vi "editDialog.vi"(0 "reference":refnum<class "InterfaceNode.lvclass">, 1 "insidePackageNode":bool, 5 "error in (no error)":errorcluster) -> (14 "reference out":refnum<class "InterfaceNode.lvclass">, 15 "changeConnection":T1, 16 "cancel":bool, 19 "error out":errorcluster)   [LabVIEW 2020, in "InterfaceNode.lvclass"]
doc: "Edit Dialog"
uses:
  <resource>/Framework/Providers/Open_GDS/UML/InterfaceNode_class/InterfaceNode.lvclass
  C:/Program Files (x86)/National Instruments/LabVIEW 2020/resource/Framework/Providers/Open_GDS/UML/ClassNode_class/ClassNode.lvclass
  C:/Program Files (x86)/National Instruments/LabVIEW 2020/resource/Framework/Providers/Open_GDS/UML/AbstractNode_class/AbstractNode.lvclass
  <resource>/Framework/Providers/Open_GDS/UML/AbstractNode_class/private/NodeConnectionStatsType.ctl
  <resource>/Framework/Providers/Open_GDS/UML/ContextHelp/ContextHelp_HelpTexts.ctl
  <resource>/Framework/Providers/Open_GDS/UML/MultiLineString_class/MultiLineString.lvclass
  <resource>/Framework/Providers/Open_GDS/UML/AbstractNode_class/AbstractNode.lvclass
  <resource>/Framework/Providers/Open_GDS/UML/ClassNode_class/ClassNode.lvclass
panel:
  in  "ShowMethods":bool caption="Show Methods"
  out "RelText":string="Relative path used"
  in  "ClassPath":path caption="LvClassPath(Optional)"
  in  "Help":bool
  in  "AddMethod":bool
  in  "connection":bool caption="Connect to Package"
  in  "Interface Name":string
  in  "Cancel Button":bool
  in  "OK Button":bool
  in  "Methods":string
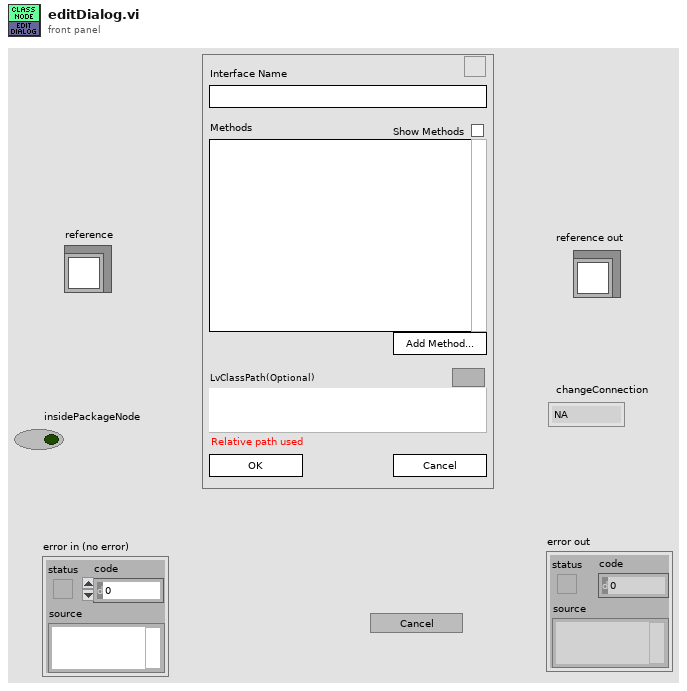
[diagram p1: front panel]
types:
  T1 = typedef "AbstractNode.lvclass/NodeConnectionStatsType.ctl" = enum16{"NA", "Connect", "DisConnect"}
  T2 = typedef "ContextHelp_HelpTexts.ctl" = enum16{"None(Hide)", "Default", "Help", "Welcome", "GettingStarted", "ClassDiagram_Help", "SequenceDiagram_Help", "UseCaseDiagram_Help", "BSelect", "BClass", "BInterface", "BPackage", "BNote", "BDependency", "BInheritance", "BInterfaceImplementation", "BAssociation", "BAggregation", "BCompAggregation", "BNoteConnector", "BObject", "BActionBar", "BCall", "BSystem", "BActor", "BUseCase", "BGeneralization", "BIncludes", "BExtends", "BUseCaseDiagramAssociation", "ClassRelationshipEdge editDialog_Bent Style", "ClassRelationshipEdge editDialog_RelationType", "ClassRelationshipEdge editDialog_Reverse association", "ClassRelationshipEdge editDialog_Start label", "ClassRelationshipEdge editDialog_Middle label", "ClassRelationshipEdge editDialog_End label", "UMLEditor reversedEngineering_Pathes", "ReversedEngineering StateReverseDialog_Help", "ReversedEngineering StateQueuedSettings_Help", "UMLEditor reversedEngineering_AddTopVIs", "UMLEditor reversedEngineering_AddClasses", "UMLEditor reversedEngineering_AddDirs", "UMLEditor reversedEngineering_Recursively", "UMLEditor reversedEngineering_Remove", "UMLEditor reversedEngineering_ClearList", "UMLEditor reversedEngineering_HideSubAss", "UMLEditor reversedEngineering_CreateTypes", "UMLEditor reversedEngineering_OnlyInheritance", "UMLEditor reversedEngineering_CreateApplication", "UMLEditor reversedEngineering_OK", "UMLEditor reversedEngineering_Cancel", "UMLEditor reversedEngineering_Help", "UMLEditor createWizardScriptFile_ScriptfilePath", "UMLEditor createWizardScriptFile_ClassPath", "UMLEditor createWizardScriptFile_Use", "UMLEditor createWizardScriptFile_PrivateDirName", "UMLEditor createWizardScriptFile_DirAppend", "UMLEditor createWizardScriptFile_Separator Character", "UMLEditor createWizardScriptFile_OK", "UMLEditor createWizardScriptFile_Cancel", "UMLEditor createWizardScriptFile_Help", "ClassNode editDialog_Class Name", "InterfaceNode editDialog_Class Name", "ClassNode editDialog_Attribute", "ClassNode editDialog_Methods", "InterfaceNode editDialog_Methods", "ClassNode editDialog_connection", "InterfaceNode editDialog_connection", "ClassNode editDialog_StereoType", "ClassNode editDialog_ShowAttrib", "ClassNode editDialog_ShowMethods", "ClassNode editDialog_ClassPath", "ClassNode editDialog_AddAttribute", "ClassNode editDialog_AddMethod", "InterfaceNode editDialog_AddMethod", "ClassNode AttributeGuide_AttributeName", "ClassNode AttributeGuide_Array?", "ClassNode AttributeGuide_Data Type", "ClassNode AttributeGuide_RefName", "ClassNode AttributeGuide_Preview", "ClassNode AttributeGuide_OK", "ClassNode AttributeGuide_Cancel", "ClassNode MethodGuide_Visibility", "ClassNode MethodGuide_Method Name", "ClassNode MethodGuide_Preview", "ClassNode MethodGuide_OK", "ClassNode MethodGuide_Cancel", "CallNode EditCallProperties_AllButtons", "ObjectNode EditObjectlProperties_AllButtons", "ActorNode EditActorProperties_AllButtons", "UseCaseRelationshipNode EditUseCaselProperties_AllButtons", "UseCaseNode EditUseCaselProperties_AllButtons", "SystemNode EditSystemProperties_AllButtons", "ReversedEngineering UpdateAttributes_AllButtons", "StateNode editDialog_AllButtons", "StateTransition editDialog_AllButtons", "ArrangeNodes Main_Picture", "ArrangeNodes Main_Zoom", "ArrangeNodes Main_Auto Zoom", "ArrangeNodes Main_shorten", "ArrangeNodes Main_Min Length", "ArrangeNodes Main_Max Length", "ArrangeNodes Main_increase", "ArrangeNodes Main_decrease", "ArrangeNodes Main_Shake", "ArrangeNodes Main", "BState", "BInitialState", "BFinalState", "BStateTransition", "StateDiagram_Help", "StateDiagram_PropertiesAllButtons", "ReversedEngineering StateReverseDialog_ClearStates", "ReversedEngineering StateReverseDialog_UseQueuedStateMachines", "ReversedEngineering StateReverseDialog_QueuedSettings", "ReversedEngineering StateReverseDialog_SearchForVIs", "ReversedEngineering StateReverseDialog_SearchCriteria", "OptionsDialog_ClassBasePath", "OptionsDialog_VIPath", "OptionsDialog_ApplicationPath", "OptionsDialog_WizDir", "OptionsDialog_IniFilePath", "OptionsDialog_DefineColors", "OptionsDialog_Help", "OptionsDialog_CreateTypes", "ClassRelationshipEdge editDialog_SplitWire"}
  T3 = enum16{"None", "TYPE", "ENUM", "ABSTRACT", "ACTOR", "GUI", "SINGLETON", "SIGNAL", "BOUNDARY", "ENTITY", "CONTROL", "LEGACY", "APPLICATION", "VI", "LVLIB"}
  T4 = typedef "ClassNode.lvclass/ObjectAttributes.ctl" = cluster{"midHeight":dbl, "botHeight":dbl, "name":refnum<class "MultiLineString.lvclass">, "attributes":refnum<class "MultiLineString.lvclass">, "methods":refnum<class "MultiLineString.lvclass">, "DEFAULT_COMPARTMENT_HEIGHT":i32, "DEFAULT_WIDTH":i32, "DEFAULT_HEIGHT":i32, "showMethods":bool, "showAttributes":bool, "ClassPath":path}
  T5 = typedef "AbstractNode.lvclass/ObjectAttributes.ctl" = cluster{"parent":refnum<class "AbstractNode.lvclass">, "children":refnum<class "AbstractNode.lvclass">[], "Hidden":bool}
  T6 = typedef "ContextHelp_ShowType.ctl" = cluster{"Header":string, "Picture":picture, "Text":string}
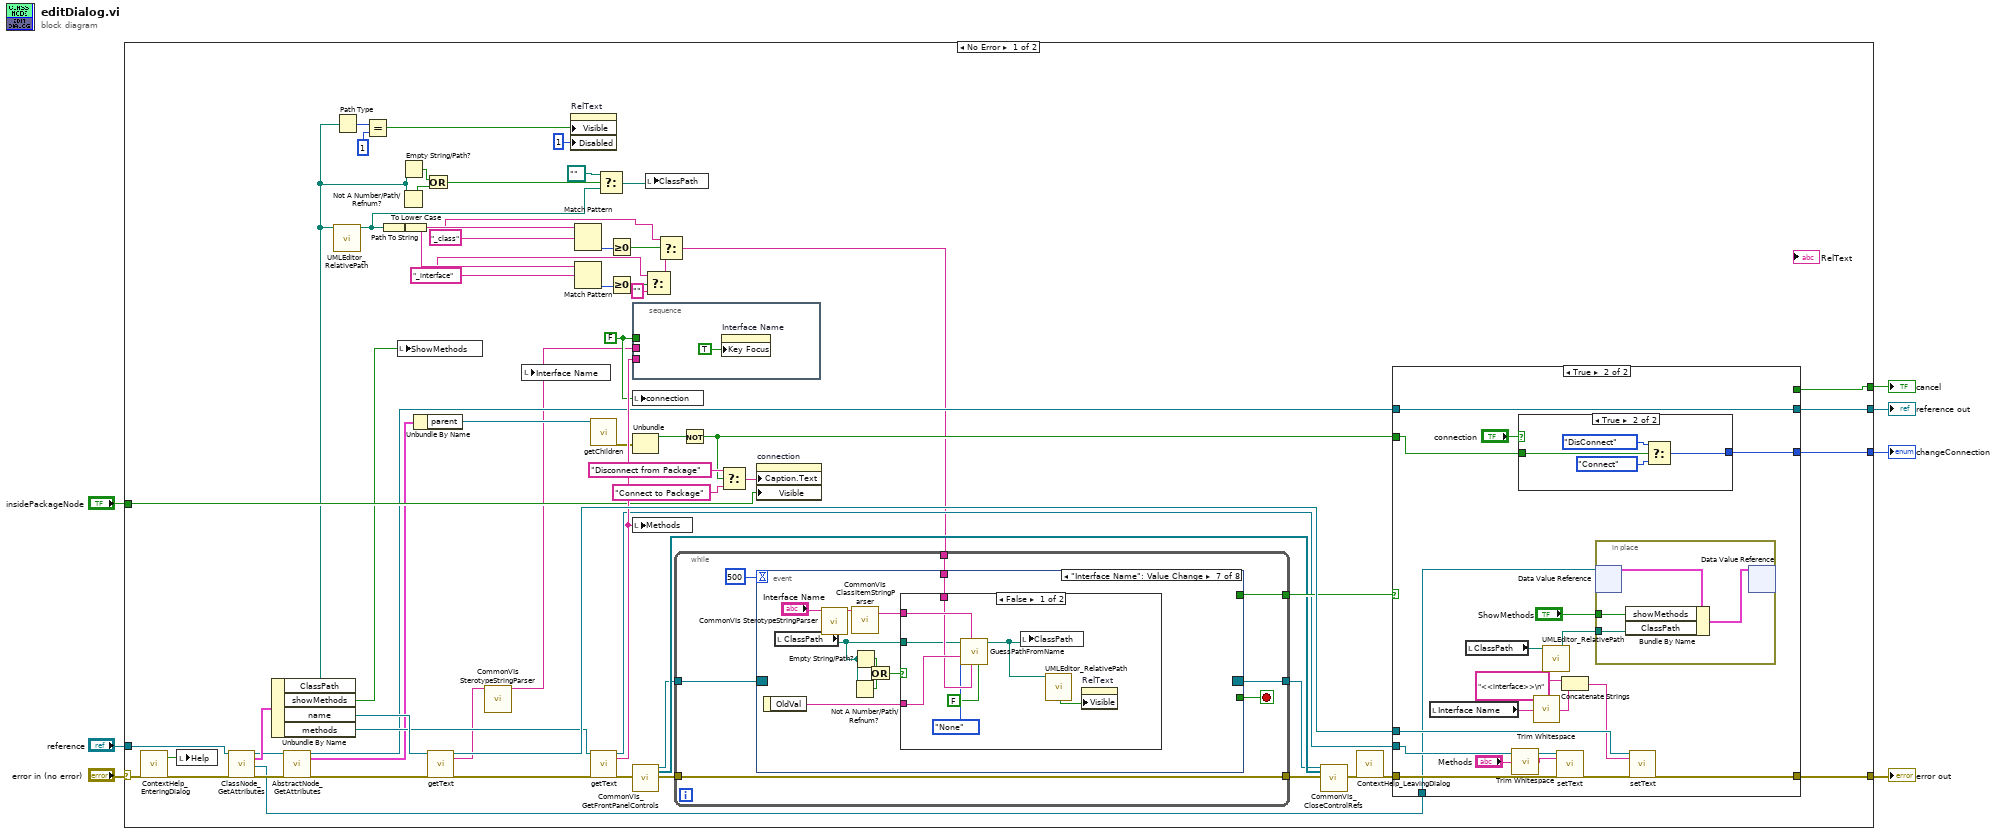
[diagram p0: block diagram]
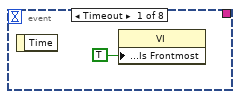
[diagram p2: hidden frame]
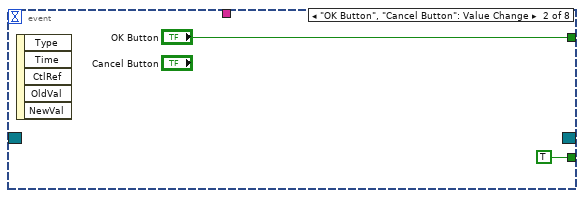
[diagram p3: hidden frame]
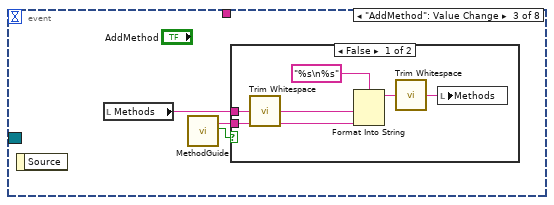
[diagram p4: hidden frame]
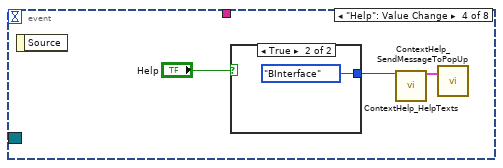
[diagram p6: hidden frame]
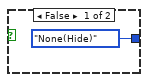
[diagram p7: hidden frame]
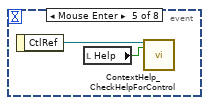
[diagram p8: hidden frame]
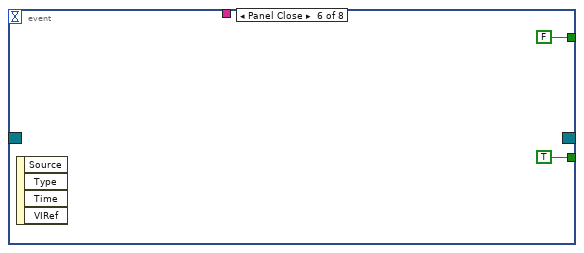
[diagram p9: hidden frame]
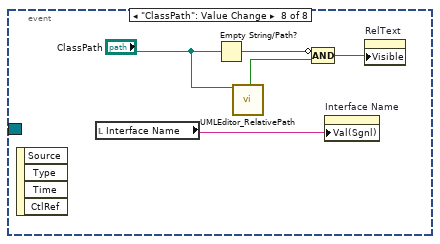
[diagram p11: hidden frame]
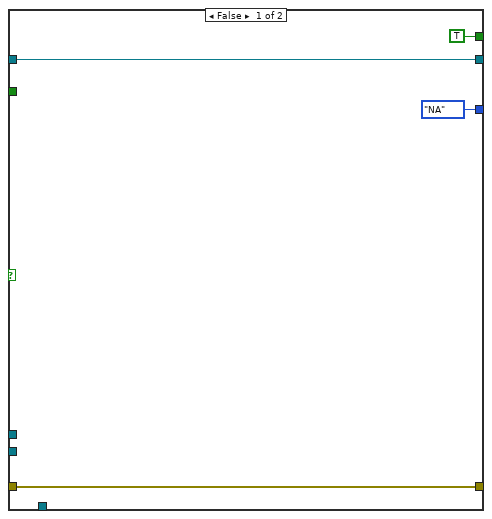
[diagram p12: hidden frame]
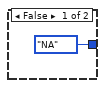
[diagram p13: hidden frame]
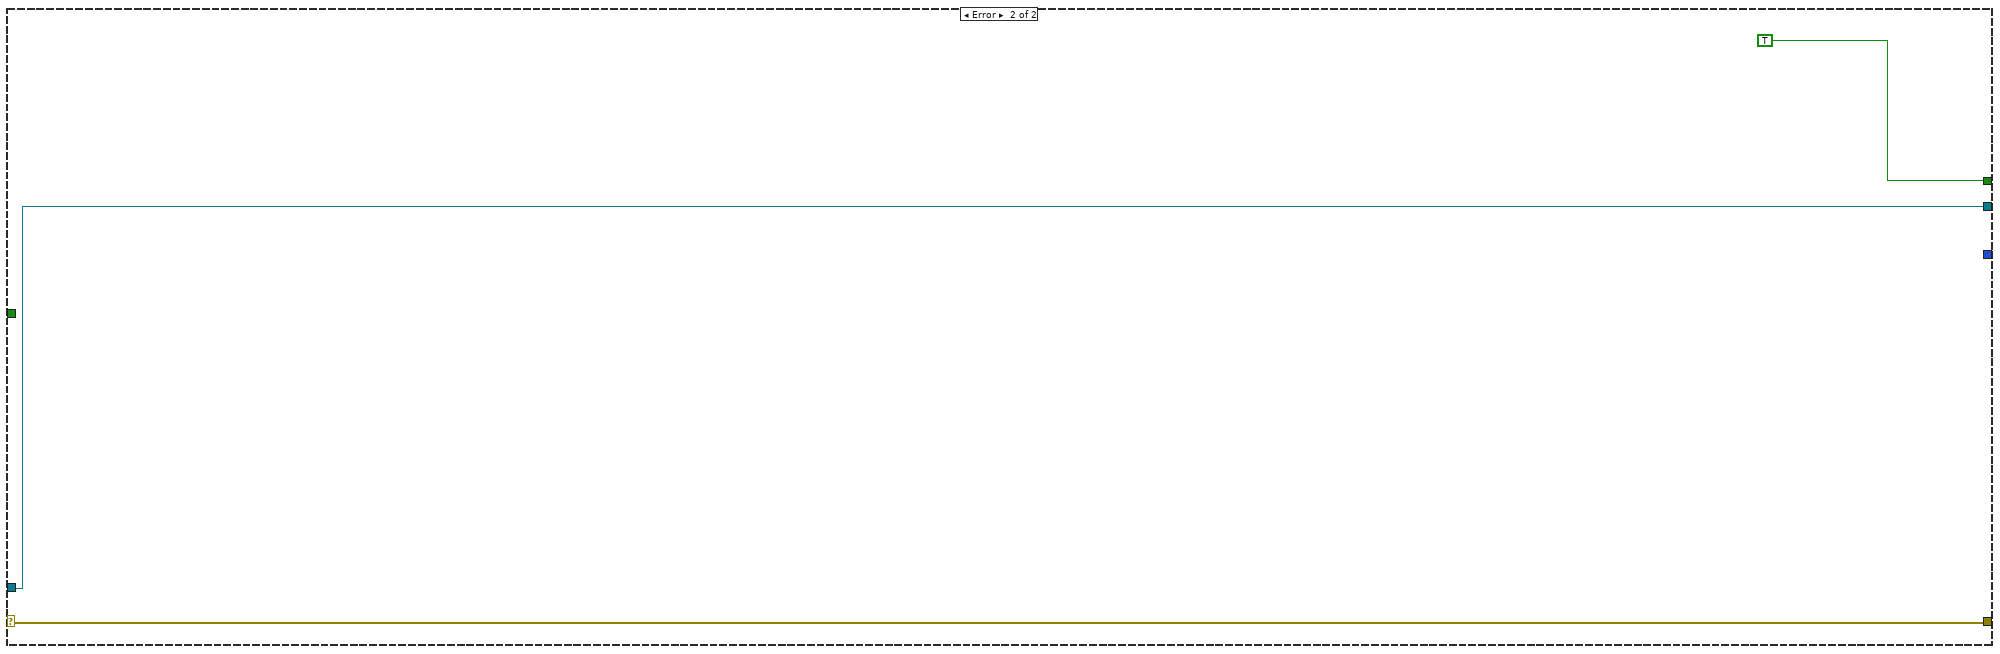
[diagram p14: hidden frame]
diagram:
  n1 = case shown="No Error" "error in (no error)" {
    selector: "error in (no error)" -> [w36 w156]
    tunnel: "reference" -> [w69 w157]
    tunnel: [w71 w156] -> w5
    tunnel: [w70 w157] -> w4
    tunnel: [w61 _] -> w3
    tunnel: "insidePackageNode" -> [w57 _]
    tunnel: [w55 TRUE ("Key Focus")] -> w1
    frame No Error {
      w14 = "_interface" ("regular expression")
      w15 = "_class" ("regular expression")
      w56 = FALSE ("connection")
      n2 = call <resource>:"ContextHelp_EnteringDialog.vi"("error in (no error)"=w36) -> ("HelpStatus"=w53:bool, "error out"=w35:errorcluster)  [unwired: 2 in, 15 out]
      n3 = local write "Help"(w53) -> ()
      n4 = call <resource>:"ClassNode_GetAttributes.vi"("reference in"=w69, "error in (no error)"=w35) -> ("reference out"=w42:refnum<class "InterfaceNode.lvclass">, "Data"=w43:T4, "DataRef"=w11:refnum<data-value>, "error out"=w41:errorcluster)  [unwired: 14 in]
      n5 = Unbundle By Name(w43) -> ("ClassPath"=w22:path, "showMethods"=w8:bool, "name"=w66:refnum<class "MultiLineString.lvclass">, "methods"=w64:refnum<class "MultiLineString.lvclass">)
      n6 = call <resource>:"AbstractNode_GetAttributes.vi"("reference in"=w42, "error in (no error)"=w41) -> ("reference out"=w39:refnum<class "InterfaceNode.lvclass">, "Data"=w38:T5, "error out"=w40:errorcluster)  [unwired: 14 in, 1 out]
      n7 = call <resource>:"UMLEditor_RelativePath.vi"("Path In"=w22) -> ("ConvertToAbsolutePath(If possible)"=w19:path)  [unwired: 1 in, 17 out]
      n8 = Path Type(1:w22) -> (0:w32:i16)
      n9 = Equal?(x=w32, y=i16 1) -> (x = y?=w30:bool)
      n10 = Path To String(path=w19) -> (string=w23:string)
      n11 = local write "ShowMethods"(w8) -> ()
      n12 = Not A Number/Path/Refnum?(number/path/refnum=w22) -> (NaN/Path/Refnum?=w28:bool)
      n13 = Empty String/Path?(string/path=w22) -> (empty?=w29:bool)
      n14 = To Lower Case(string=w23) -> (all lower case string=w20:string)
      n15 = Unbundle By Name(w38) -> ("parent"=w45:refnum<class "AbstractNode.lvclass">)
      n16 = Or(x=w29, y=w28) -> (x .or. y?=w26:bool)
      n17 = call-dynamic "getText.vi"("reference"=w66, "error in (no error)"=w40) -> ("reference out"=w68:refnum<class "MultiLineString.lvclass">, "text"=w10:string, "error out"=w62:errorcluster)  [unwired: 15 in]
      n18 = call <resource>:"CommonVIs SterotypeStringParser.vi"("SterotypeStringIn"=w10) -> ("Name"=w9:string)  [unwired: 18 out]
      n19 = local write "Interface Name"(w9) -> ()
      n20 = property on="RelText" class="Str"("Visible"=w30, "Disabled"=u8 1) -> ()  [unwired: 2 in, 2 out]
      n21 = Match Pattern(string=w20, regular expression=w15) -> (offset past match=w24:i32)  [unwired: 1 in, 3 out]
      n22 = Match Pattern(string=w20, regular expression=w14) -> (offset past match=w21:i32)  [unwired: 1 in, 3 out]
      n23 = call-dynamic "getChildren.vi"("reference"=w45) -> ("error out"=w47:errorcluster)  [unwired: 15 in, 3 out]
      n24 = call-dynamic "getText.vi"("reference"=w64, "error in (no error)"=w62) -> ("reference out"=w63:refnum<class "MultiLineString.lvclass">, "text"=w65:string, "error out"=w37:errorcluster)  [unwired: 15 in]
      n25 = Select(t=path "", s=w26, f=w19) -> (s? t:f=w25:path)
      n26 = Greater Or Equal To 0?(x=w24) -> (x >= 0?=w18:bool)
      n27 = Greater Or Equal To 0?(x=w21) -> (x >= 0?=w16:bool)
      n28 = stacked-sequence {
        tunnel: w9 -> [_]
        tunnel: w65 -> [_]
        tunnel: w56 -> [_]
        frame #0 {
          n29 = property on="Interface Name" class="Str"("Key Focus"=TRUE) -> ()  [unwired: 2 in, 2 out]
        }
      }
      n30 = local write "connection"(w56) -> ()
      n31 = Unbundle(w47) -> ("status"=w46:bool)  [unwired: 2 out]
      n32 = local write "Methods"(w65) -> ()
      n33 = call <resource>:"CommonVIs_GetFrontPanelControls.vi"("error in (no error)"=w37) -> ("Event Registration Refnum"=w49:refnum<event-registration>, "ControlRefs"=w50:refnum<vi>[], "error out"=w54:errorcluster)  [unwired: 1 in, 15 out]
      n34 = local write "ClassPath"(w25) -> ()
      n35 = Select(t=w14, s=w16, f="") -> (s? t:f=w17:string)
      n36 = Select(t=w15, s=w18, f=w17) -> (s? t:f=w12:string)
      n37 = while {
        tunnel: [w78] -> w67
        tunnel: [w75] -> w52
        tunnel: w54 -> [w75]
        tunnel: w49 -> [w74]
        tunnel: [w73] -> w48
        tunnel: w12 -> [w72]
        stop <- w76 stop-if-true
        n38 = event shown="[6] \"Interface Name\": Value Change" {
          selector: w74 -> [_ _ _ _ _ _ _ _]
          dyn-events: [_ _ _ _ _ _ _ _] -> w73
          timeout: 500 -> [_ _ _ _ _ _ _ _]
          tunnel: [_ "OK Button" _ _ _ FALSE ("OK Button") _ _] -> w78
          tunnel: [_ TRUE _ _ _ TRUE ("Front Panel Window:Is Frontmost") _ _] -> w76
          tunnel: w72 -> [_ _ _ _ _ _ w104 _]
          event Timeout {
            n39 = event-data() -> ()  [unwired: 2 out]
            n40 = property class="VI"("Front Panel Window:Is Frontmost"=TRUE) -> ()  [unwired: 2 in, 2 out]
          }
          event "OK Button", "Cancel Button": Value Change {
            n41 = event-data() -> ()  [unwired: 6 out]
          }
          event "AddMethod": Value Change {
            n42 = event-data() -> ()  [unwired: 2 out]
            n43 = local read "Methods"() -> (w84:string)
            n44 = call <resource>:"MethodGuide.vi"() -> ("Preview"=w83:string, "Canceled"=w82:bool)  [unwired: 1 in, 17 out]
            n45 = case shown="False" w82 {
              tunnel: w84 -> [w90 _]
              tunnel: w83 -> [w87 _]
              frame False {
                n46 = call <vilib>:"Trim Whitespace.vi"("string"=w90) -> ("trimmed string"=w88:string)  [unwired: 1 in]
                n47 = Format Into String(format string="%s\n%s", w88, w87) -> (resulting string=w86:string)  [unwired: 2 in, 1 out]
                n48 = call <vilib>:"Trim Whitespace.vi"("string"=w86) -> ("trimmed string"=w85:string)  [unwired: 1 in]
                n49 = local write "Methods"(w85) -> ()
              }
              frame True {
              }
            }
          }
          event "Help": Value Change {
            n50 = event-data() -> ()  [unwired: 2 out]
            n51 = case shown="True" "Help" {
              tunnel: [ContextHelp_HelpTexts."None(Hide)" ("HelpText") ContextHelp_HelpTexts."BInterface" ("HelpText")] -> w92
              frame False {
              }
              frame True {
              }
            }
            n52 = call <resource>:"ContextHelp_HelpTexts.vi"("HelpText (enum or string)"=w92) -> ("HelpOut"=w93:T6)  [unwired: 18 out]
            n53 = call <resource>:"ContextHelp_SendMessageToPopUp.vi"("PopUpMessage"=w93) -> ()  [unwired: 2 in, 17 out]
          }
          event Mouse Enter {
            n54 = event-data() -> ("CtlRef"=w97:refnum<vi>)  [unwired: 1 out]
            n55 = local read "Help"() -> (w96:bool)
            n56 = call <resource>:"ContextHelp_CheckHelpForControl.vi"("Ctl Refnum"=w97, "Help"=w96) -> ()  [unwired: 1 in, 17 out]
          }
          event Panel Close {
            n57 = event-data() -> ()  [unwired: 5 out]
          }
          event "Interface Name": Value Change {
            n58 = event-data() -> ("OldVal"=w105:string)  [unwired: 1 out]
            n59 = local read "ClassPath"() -> (w101:path)
            n60 = call <resource>:"CommonVIs SterotypeStringParser.vi"("SterotypeStringIn"="Interface Name") -> ("Name"=w108:string)  [unwired: 18 out]
            n61 = Not A Number/Path/Refnum?(number/path/refnum=w101) -> (NaN/Path/Refnum?=w103:bool)
            n62 = call <resource>:"CommonVIs ClassItemStringParser.vi"("ClassItemNameIn"=w108) -> ("Name"=w106:string)  [unwired: 18 out]
            n63 = Empty String/Path?(string/path=w101) -> (empty?=w102:bool)
            n64 = Or(x=w102, y=w103) -> (x .or. y?=w100:bool)
            n65 = case shown="False" w100 {
              tunnel: w106 -> [w116 _]
              tunnel: w105 -> [w115 _]
              tunnel: w104 -> [w114 _]
              tunnel: w101 -> [w109 _]
              frame False {
                n66 = call <resource>:"GuessPathFromName.vi"("Don'tAppendName"=FALSE, "FolderSuffix"=w114, "NewName"=w116, "OldName"=w115, "Stereo Type"=T3."None", "PathIn"=w109) -> ("File Path"=w112:path)  [unwired: 5 in]
                n67 = local write "ClassPath"(w112) -> ()
                n68 = call <resource>:"UMLEditor_RelativePath.vi"("Path In"=w112) -> ("ConvertedToARelativePath"=w111:bool)  [unwired: 1 in, 17 out]
                n69 = property on="RelText" class="Str"("Visible"=w111) -> ()  [unwired: 2 in, 2 out]
              }
              frame True {
              }
            }
          }
          event "ClassPath": Value Change {
            n70 = event-data() -> ()  [unwired: 5 out]
            n71 = local read "Interface Name"() -> (w117:string)
            n72 = Empty String/Path?(string/path="ClassPath") -> (empty?=w121:bool)
            n73 = call <resource>:"UMLEditor_RelativePath.vi"("Path In"="ClassPath") -> ("ConvertedToARelativePath"=w120:bool)  [unwired: 1 in, 17 out]
            n74 = Compound Arithmetic op=AND(invert w121, w120) -> (w118:bool)
            n75 = property on="Interface Name" class="Str"("Val(Sgnl)"=w117) -> ()  [unwired: 2 in, 2 out]
            n76 = property on="RelText" class="Str"("Visible"=w118) -> ()  [unwired: 2 in, 2 out]
          }
        }
      }
      n77 = Not(x=w46) -> (.not. x?=w44:bool)
      n78 = Select(t="Disconnect from Package", s=w44, f="Connect to Package") -> (s? t:f=w60:string)
      n79 = property on="connection" class="Bool (strict)"("Caption.Text"=w60, "Visible"=w57) -> ()  [unwired: 2 in, 2 out]
      n80 = call <resource>:"CommonVIs_CloseControlRefs.vi"("Event Registration Refnum"=w48, "ControlRefs"=w50, "error in (no error)"=w52) -> ("error out"=w51:errorcluster)  [unwired: 16 out]
      n81 = call <resource>:"ContextHelp_LeavingDialog.vi"("error in (no error)"=w51) -> ("error out"=w34:errorcluster)  [unwired: 2 in, 16 out]
      n82 = case shown="True" w67 {
        tunnel: [w124 w139] -> w71
        tunnel: [w125 w140] -> w70
        tunnel: w39 -> [w125 w140]
        tunnel: w68 -> [_ w144]
        tunnel: w63 -> [_ w143]
        tunnel: w34 -> [w124 w142]
        tunnel: [enum16{"NA", "Connect", "DisConnect"}."NA" ("changeConnection") w137] -> w61
        tunnel: w44 -> [_ w136]
        tunnel: [TRUE ("Key Focus") _] -> w55
        tunnel: w11 -> [_ w134]
        frame False {
        }
        frame True {
          n83 = local read "Interface Name"() -> (w135:string)
          n84 = local read "ClassPath"() -> (w133:path)
          n85 = call <vilib>:"Trim Whitespace.vi"("string"="Methods") -> ("trimmed string"=w131:string)  [unwired: 1 in]
          n86 = case shown="True" "connection" {
            tunnel: [enum16{"NA", "Connect", "DisConnect"}."NA" ("changeConnection") w152] -> w137
            tunnel: w136 -> [_ w153]
            frame False {
            }
            frame True {
              n87 = Select(t=enum16{"NA", "Connect", "DisConnect"}."DisConnect" ("changeConnection"), s=w153, f=enum16{"NA", "Connect", "DisConnect"}."Connect" ("changeConnection")) -> (s? t:f=w152:enum16{"NA", "Connect", "DisConnect"})
            }
          }
          n88 = call <vilib>:"Trim Whitespace.vi"("string"=w135) -> ("trimmed string"=w128:string)  [unwired: 1 in]
          n89 = call <resource>:"UMLEditor_RelativePath.vi"("Path In"=w133) -> ("ConvertToRelativePath(If possible)"=w132:path)  [unwired: 1 in, 17 out]
          n90 = call-dynamic "setText.vi"("reference"=w143, "text"=w131, "error in (no error)"=w142) -> ("error out"=w141:errorcluster)  [unwired: 15 in, 1 out]
          n91 = Concatenate Strings("<<interface>>\n" ("text"), w128) -> (w127:string)
          n92 = in-place {
            in-place-border: w132 -> [w147]
            in-place-border: "ShowMethods" -> [w145]
            n93 = in-place-dvr #1(w134) -> (w146:T4)  [unwired: 1 out]
            n94 = Bundle By Name(cluster=w146, "showMethods"=w145, "ClassPath"=w147) -> (w148:T4)
            n95 = in-place-dvr #1(w148) -> ()  [unwired: 2 out]
          }
          n96 = call-dynamic "setText.vi"("reference"=w144, "text"=w127, "error in (no error)"=w141) -> ("error out"=w139:errorcluster)  [unwired: 15 in, 1 out]
        }
      }
    }
    frame Error {
    }
  }
  "reference out" <- w4
  "error out" <- w5
  "changeConnection" <- w3
  "cancel" <- w1
